vi "FX232_485_BRWR.vi"(5 "延时":u8 max=150 step=10, 6 "数量":u8=1, 7 "PLC站号":u8=1, 8 "error in (no error)":errorcluster caption="错误输入（无错误）", 9 "地址":string, 10 "命令":string(combo), 11 "Port":refnum<visa-resource-name>) -> (0 "error out":errorcluster caption="错误输出", 1 "Value":string, 2 "匹配":bool, 3 "PortOut":refnum<visa-resource-name>)   [LabVIEW 2025]
uses:
  <vilib>/Utility/error.llb/Trim Whitespace One-Sided.vi
panel:
  out "连接的字符串":string
  out "Buff":string
  # "X,Y,D,S,M"
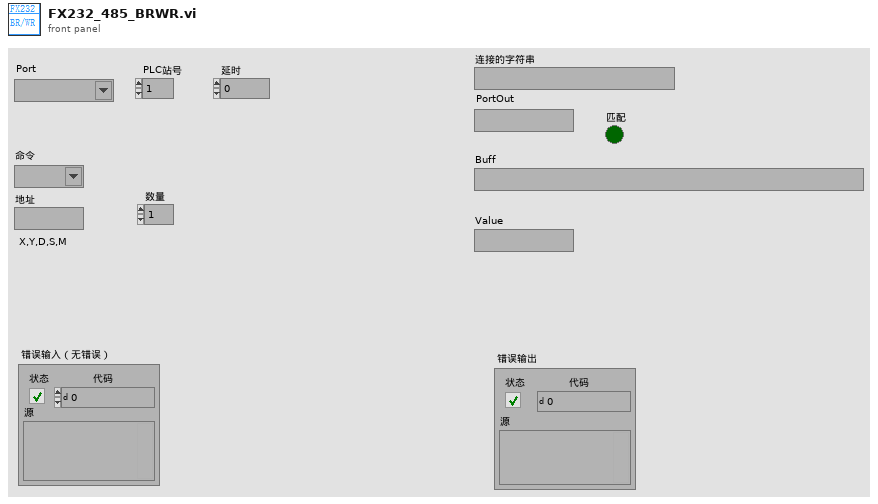
[diagram p1: front panel]
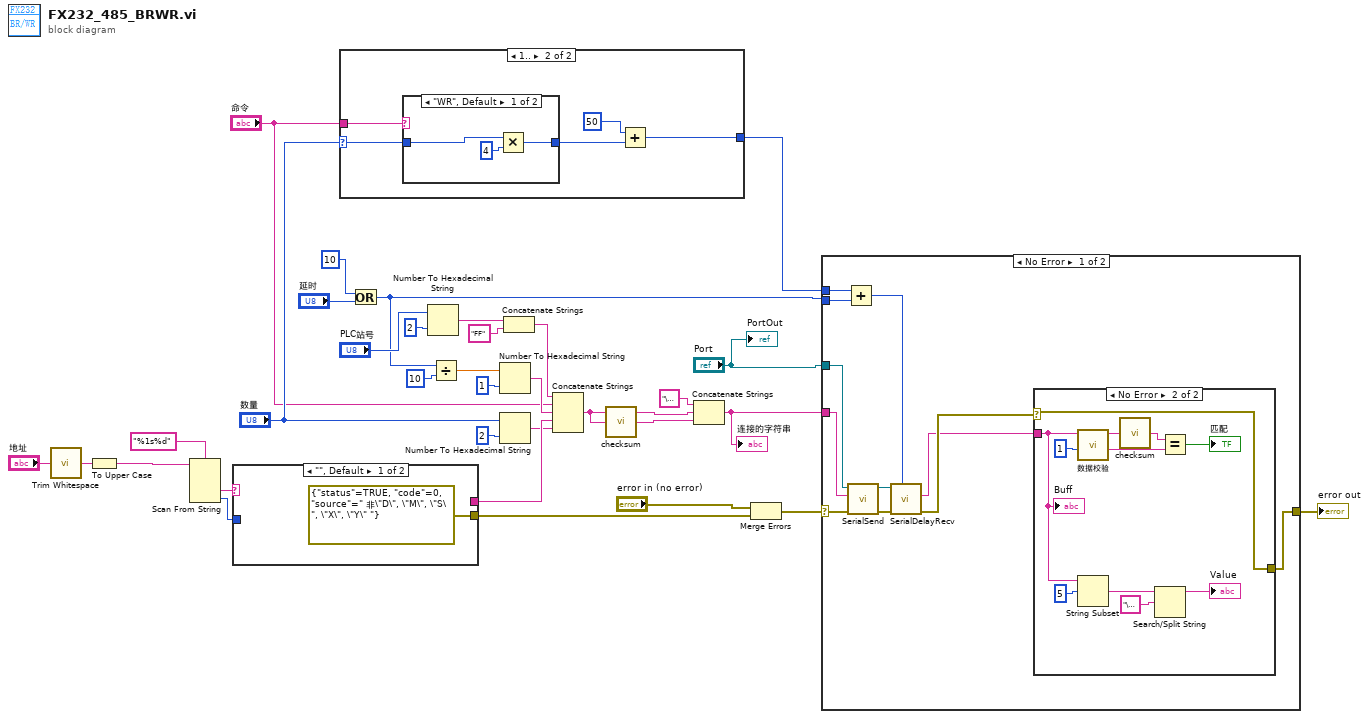
[diagram p0: block diagram]
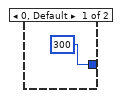
[diagram p2: hidden frame]
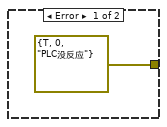
[diagram p4: hidden frame]
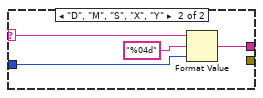
[diagram p6: hidden frame]
diagram:
  n1 = call <vilib>:"Trim Whitespace.vi"("string"="地址") -> ("trimmed string"=w29:string)  [unwired: 1 in]
  n2 = To Upper Case(1:w29) -> (0:w31:string)
  n3 = Scan From String(format string="%1s%d" ("格式字符串"), input string=w31) -> (output 1=w32:string, output 2=w28:i32)  [unwired: 4 in, 3 out]
  n4 = case shown="\"\", Default" w32 {
    selector: w32 -> [_ w38]
    tunnel: w28 -> [_ w37]
    tunnel: [errorcluster {"status"=TRUE, "code"=0, "source"=" 非\"D\", \"M\", \"S\", \"X\", \"Y\" "} ("error in (no error)") _] -> w5
    tunnel: [_ w36] -> w21
    frame "", Default {
    }
    frame "D", "M", "S", "X", "Y" {
      n5 = Format Value(string ("")=w38, format string="%04d" ("格式字符串"), value (0)=w37) -> (output string=w36:string)
    }
  }
  n6 = case shown="1.." "数量" {
    selector: "数量" -> [_ w41]
    tunnel: [300 w43] -> w8
    tunnel: "命令" -> [_ w42]
    frame 0, Default {
    }
    frame 1.. {
      n7 = case shown="\"WR\", Default" w42 {
        tunnel: w41 -> [w47 w48]
        tunnel: [w45 w48] -> w40
        frame "WR", Default {
          n8 = Multiply(x=w47, y=u8 4) -> (x*y=w45:u8)
        }
        frame "BR" {
        }
      }
      n9 = Add(x=50, y=w40) -> (x+y=w43:i32)
    }
  }
  n10 = Or(x=u8 10, y="延时") -> (x .or. y?=w2:u8)
  n11 = Number To Hexadecimal String(1:i16 2 ("宽度(-)"), 2:"PLC站号") -> (0:w19:string)
  n12 = Divide(x=w2, y=10) -> (x/y=w23:dbl)
  n13 = Number To Hexadecimal String(1:i16 1 ("宽度(-)"), 2:w23) -> (0:w18:string)
  n14 = Number To Hexadecimal String(1:i16 2 ("宽度(-)"), 2:"数量") -> (0:w11:string)
  n15 = Concatenate Strings(w19, "FF" ("字符串")) -> (w16:string)
  n16 = Concatenate Strings(w16, "命令", w18, w21, w11) -> (w13:string)
  n17 = call "checksum.vi"("buff"=w13) -> ("checksum"=w12:string)  [unwired: 4 in]
  n18 = Concatenate Strings("\u0005" ("字符串"), w13, w12) -> (w22:string)
  "连接的字符串" <- w22
  n19 = Merge Errors("error in (no error)", w5) -> (w4:errorcluster)
  n20 = case shown="No Error" w4 {
    selector: w4 -> [w57 w72]
    tunnel: w22 -> [w59 _]
    tunnel: "Port" -> [w58 _]
    tunnel: [w56 w72] -> w27
    tunnel: w2 -> [w55 _]
    tunnel: w8 -> [w54 _]
    frame No Error {
      n21 = Add(x=w54, y=w55) -> (x+y=w53:i32)
      n22 = call "SerialSend.vi"("error in (no error)"=w57, "SendData"=w59, "PORT"=w58) -> ("error out"=w51:errorcluster, "PORT out"=w52:refnum<visa-resource-name>)  [unwired: 6 in, 1 out]
      n23 = call "SerialDelayRecv.vi"("Timeout"=w53, "error in (no error)"=w51, "Port"=w52) -> ("error out"=w50:errorcluster, "Buff"=w49:string)  [unwired: 6 in, 1 out]
      n24 = case shown="No Error" w50 {
        selector: w50 -> [_ w61]
        tunnel: [errorcluster {"status"=TRUE, "code"=0, "source"="PLC没反应"} ("错误常量") w61] -> w56
        tunnel: w49 -> [_ w63]
        frame Error {
        }
        frame No Error {
          n25 = call "数据校验.vi"("偏移量(0)"=1, "字符串"=w63) -> ("校验字符串"=w64:string, "数据字符串"=w65:string)  [unwired: 8 in]
          n26 = String Subset(string=w63, offset (0)=5 ("偏移量(0)")) -> (substring=w68:string)  [unwired: 1 in]
          n27 = call "checksum.vi"("buff"=w65) -> ("checksum"=w69:string)  [unwired: 4 in]
          n28 = Search/Split String(string=w68, search string/char (-)="\u0003") -> (substring before match=→"Value":string)  [unwired: 1 in, 2 out]
          n29 = Equal?(x=w69, y=w64) -> (x = y?=→"匹配":bool)
          "Buff" <- w63
        }
      }
    }
    frame Error {
    }
  }
  "error out" <- w27
  "PortOut" <- "Port"
